vi "LHF.DB.MongoDB.vi"() -> ()   [LabVIEW 2013]
uses:
  src/LHF.DB.Mongo.lvclass
panel:
  out "Document":variant
  out "Document Part":bool
  out "error out":errorcluster
  out "Nested Documents":bool
  out "Update (Existent Field)":bool
  out "Inserted":bool
  out "Update (New Field)":bool
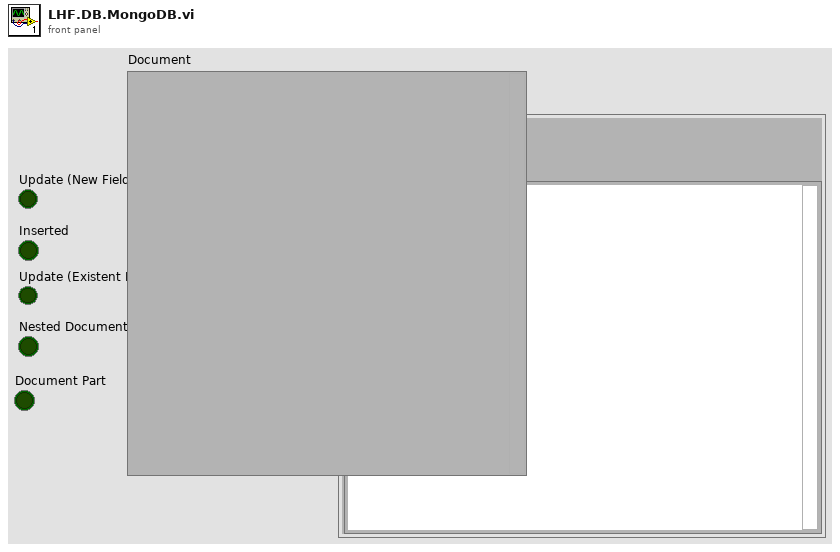
[diagram p1: front panel]
types:
  T1 = cluster{"email":string, "name":string, "status":i32, "CrazyData":cluster{"CrazyArray":cluster{"MyArray":i32[], "MyString":string, "SubSubClust":cluster{"MyArray":i32[], "MyString":string}}[][]}}
  T2 = cluster{"email":string, "name":string, "status":i32}
  T3 = cluster{"CrazyArray":cluster{"MyArray":i32[], "MyString":string, "SubSubClust":cluster{"MyArray":i32[], "MyString":string}}[][]}
  T4 = cluster{"name":string, "CrazyData":cluster{"CrazyArray":cluster{"MyArray":i32[], "MyString":string, "SubSubClust":cluster{"MyArray":i32[], "MyString":string}}[][]}}
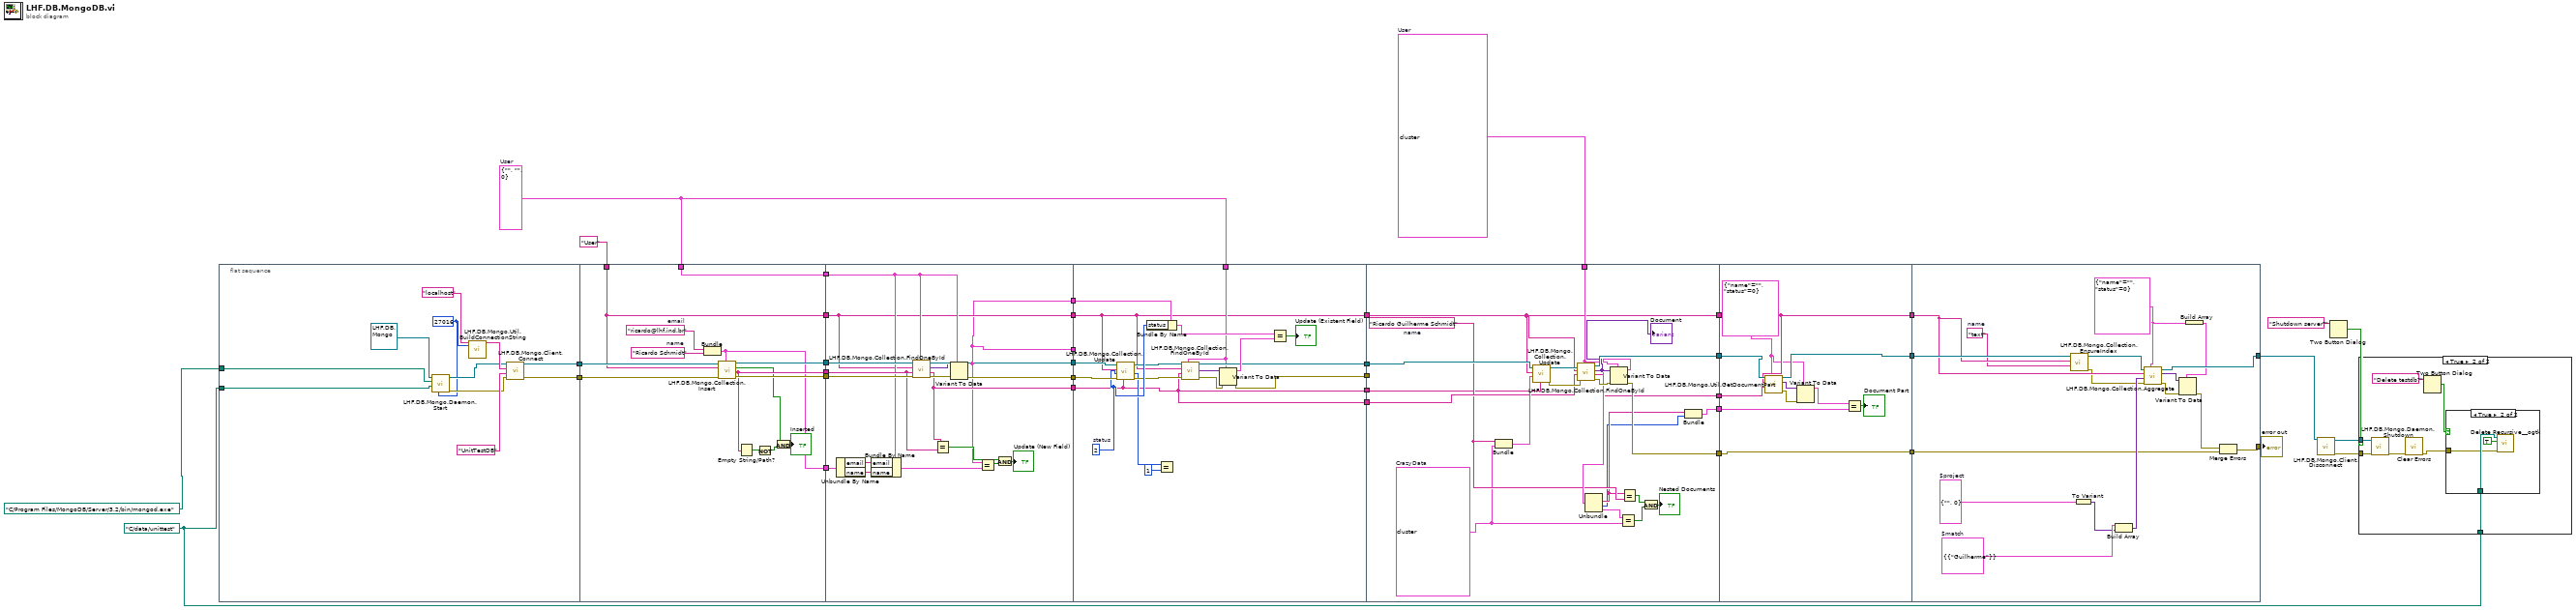
[diagram p0: block diagram]
diagram:
  w11 = path "C:/data/unittest" ("data folder")
  w17 = T1 {"email"="ricardo@lhf.ind.br", "name"="Ricardo Guilherme Schmidt", "status"=2, "CrazyData"={"CrazyArray"=[[{"MyArray"=[1, 2, 3], "MyString"="MyText", "SubSubClust"={"MyArray"=[3, 4, 5], "MyString"="MyText2"}}, {"MyArray"=[7, 8, 9], "MyString"="MyText3", "SubSubClust"={"MyArray"=[10, 11, 12], "MyString"="MyText4"}}]]}}  # User
  w22 = T2 {"email"="", "name"="", "status"=0}  # User
  n1 = flat-sequence {
    tunnel: [w46] -> w38
    tunnel: [w45] -> w37
    tunnel: w11 -> [w40]
    tunnel: path "C:/Program Files/MongoDB/Server/3.2/bin/mongod.exe" ("mongod path") -> [w39]
    tunnel: w38 -> [w61]
    tunnel: w37 -> [w63]
    tunnel: [w62] -> w36
    tunnel: [w60] -> w35
    tunnel: "User" ("database") -> [w59]
    tunnel: w22 -> [w56]
    tunnel: [w55] -> w31
    tunnel: [w59] -> w30
    tunnel: [w56] -> w29
    tunnel: [w51] -> w28
    tunnel: w36 -> [w80]
    tunnel: w35 -> [w81]
    tunnel: [w79] -> w34
    tunnel: [w76] -> w33
    tunnel: w31 -> [w75]
    tunnel: w30 -> [w66]
    tunnel: w29 -> [w73]
    tunnel: w28 -> [w74]
    tunnel: [w66] -> w27
    tunnel: [w65] -> w26
    tunnel: [w64] -> w24
    tunnel: [w64] -> w23
    tunnel: w34 -> [w98]
    tunnel: w33 -> [w99]
    tunnel: w27 -> [w83]
    tunnel: w26 -> [w82]
    tunnel: [w87] -> w25
    tunnel: w24 -> [_]
    tunnel: w23 -> [w97]
    tunnel: w22 -> [w86]
    tunnel: [w88] -> w20
    tunnel: [w82] -> w19
    tunnel: [w83] -> w18
    tunnel: [w82] -> w16
    tunnel: w25 -> [_]
    tunnel: w20 -> [w122]
    tunnel: w19 -> [w113]
    tunnel: w18 -> [w105]
    tunnel: w17 -> [w116]
    tunnel: [w118] -> w10
    tunnel: [w114] -> w8
    tunnel: [w105] -> w7
    tunnel: w16 -> [w104]
    tunnel: [w103] -> w5
    tunnel: [w100] -> w4
    tunnel: w10 -> [w133]
    tunnel: [w132] -> w9
    tunnel: w8 -> [w123]
    tunnel: w7 -> [w131]
    tunnel: [w131] -> w6
    tunnel: w5 -> [w130]
    tunnel: w4 -> [w125]
    tunnel: [w123] -> w1
    tunnel: [w149] -> w21
    tunnel: w9 -> [w150]
    tunnel: w6 -> [w139]
    tunnel: [w135] -> w13
    tunnel: w1 -> [w134]
    frame #0 {
      w41 = u32 27016 ("Port (27017)")
      n2 = call-dynamic "LHF.DB.Mongo.Daemon.Start.vi"("Port (27017)"=w41, "data folder"=w40, "mongod path"=w39, "LHF.DB.Mongo in"=refnum<class "LHF.DB.Mongo.lvclass"> refnum) -> ("error out"=w42:errorcluster, "LHF.DB.Mongo out"=w44:refnum<class "LHF.DB.Mongo.lvclass">)  [unwired: 6 in]
      n3 = call "LHF.DB.Mongo.Util.BuildConnectionString.vi"("host"="localhost", "port"=w41) -> ("connectionString"=w49:string)  [unwired: 17 in]
      n4 = call-dynamic "LHF.DB.Mongo.Client.Connect.vi"("error in (no error)"=w42, "database"="UnitTestDB", "url"=w49, "LHF.DB.Mongo in"=w44) -> ("error out"=w45:errorcluster, "LHF.DB.Mongo out"=w46:refnum<class "LHF.DB.Mongo.lvclass">)  [unwired: 6 in]
    }
    frame #1 {
      w57 = "Ricardo Schmidt"  # name
      w58 = "ricardo@lhf.ind.br"  # email
      n5 = Bundle("email"=w58, "name"=w57) -> (w51:cluster{"email":string, "name":string})  [unwired: 1 in]
      n6 = call-dynamic "LHF.DB.Mongo.Collection.Insert.vi"("Document"=w51, "error in (no error)"=w63, "Collection"=w59, "LHF.DB.Mongo"=w61) -> ("error out"=w62:errorcluster, "_id"=w55:string, "Ok"=w52:bool, "LHF.DB.Mongo out"=w60:refnum<class "LHF.DB.Mongo.lvclass">)  [unwired: 4 in]
      n7 = Empty String/Path?(string/path=w55) -> (empty?=w54:bool)
      n8 = Not(x=w54) -> (.not. x?=w53:bool)
      n9 = And(x=w52, y=w53) -> (x .and. y?=→"Inserted":bool)
    }
    frame #2 {
      n10 = Unbundle By Name(w74) -> ("email"=w72:string, "name"=w71:string)
      n11 = Bundle By Name(cluster=w73, "email"=w72, "name"=w71) -> (w70:T2)
      n12 = call-dynamic "LHF.DB.Mongo.Collection.FindOneById.vi"("type"=w73, "error in (no error)"=w80, "_id"=w75, "Collection"=w66, "LHF.DB.Mongo in"=w81) -> ("error out"=w78:errorcluster, "_id"=w65:string, "Document"=w77:variant, "LHF.DB.Mongo out"=w79:refnum<class "LHF.DB.Mongo.lvclass">)  [unwired: 3 in]
      n13 = Equal?(x=w65, y=w75) -> (x = y?=w69:bool)
      n14 = Variant To Data(error in=w78, type=w73, Variant=w77) -> (data=w64:T2, error out=w76:errorcluster)
      n15 = Equal?(x=w64, y=w70) -> (x = y?=w68:bool)
      n16 = And(x=w69, y=w68) -> (x .and. y?=→"Update (New Field)":bool)
    }
    frame #3 {
      w96 = 2  # status
      n17 = call-dynamic "LHF.DB.Mongo.Collection.Update.vi"("Query"=w82, "error in (no error)"=w99, "Update"=w96, "Collection"=w83, "LHF.DB.Mongo in"=w98) -> ("error out"=w94:errorcluster, "DocumentsAffected"=w85:i64, "LHF.DB.Mongo out"=w95:refnum<class "LHF.DB.Mongo.lvclass">)  [unwired: 3 in, 1 out]
      n18 = Bundle By Name(cluster=w97, "status"=w96) -> (w90:T2)
      n19 = Equal?(x=w85, y=i64 1) -> ()  [unwired: 1 out]
      n20 = call-dynamic "LHF.DB.Mongo.Collection.FindOneById.vi"("type"=w86, "error in (no error)"=w94, "_id"=w82, "Collection"=w83, "LHF.DB.Mongo in"=w95) -> ("error out"=w92:errorcluster, "Document"=w93:variant, "LHF.DB.Mongo out"=w88:refnum<class "LHF.DB.Mongo.lvclass">)  [unwired: 3 in, 1 out]
      n21 = Variant To Data(error in=w92, type=w86, Variant=w93) -> (data=w91:T2, error out=w87:errorcluster)
      n22 = Equal?(x=w90, y=w91) -> (x = y?=→"Update (Existent Field)":bool)
    }
    frame #4 {
      w109 = T3 {"CrazyArray"=[[{"MyArray"=[1, 2, 3], "MyString"="MyText", "SubSubClust"={"MyArray"=[3, 4, 5], "MyString"="MyText2"}}, {"MyArray"=[7, 8, 9], "MyString"="MyText3", "SubSubClust"={"MyArray"=[10, 11, 12], "MyString"="MyText4"}}], [{"MyArray"=[1, 2, 3], "MyString"="MyText", "SubSubClust"={"MyArray"=[1, 2, 3], "MyString"="MyText"}}, {"MyArray"=[1, 2, 3], "MyString"="MyText", "SubSubClust"={"MyArray"=[1, 2, 3], "MyString"="MyText"}}]]}  # CrazyData
      w111 = "Ricardo Guilherme Schmidt"  # name
      n23 = Bundle("name"=w111, "CrazyData"=w109) -> (w121:T4)  [unwired: 1 in]
      n24 = call-dynamic "LHF.DB.Mongo.Collection.Update.vi"("Query"=w104, "Update"=w121, "Collection"=w105, "LHF.DB.Mongo in"=w122) -> ("error out"=w120:errorcluster, "LHF.DB.Mongo out"=w119:refnum<class "LHF.DB.Mongo.lvclass">)  [unwired: 4 in, 2 out]
      n25 = call-dynamic "LHF.DB.Mongo.Collection.FindOneById.vi"("type"=w116, "error in (no error)"=w120, "_id"=w113, "Collection"=w105, "LHF.DB.Mongo in"=w119) -> ("error out"=w115:errorcluster, "_id"=w103:string, "Document"=w117:variant, "LHF.DB.Mongo out"=w118:refnum<class "LHF.DB.Mongo.lvclass">)  [unwired: 3 in]
      "Document" <- w117
      n26 = Variant To Data(error in=w115, type=w116, Variant=w117) -> (data=w112:T1, error out=w114:errorcluster)
      n27 = Unbundle(w112) -> ("name"=w102:string, "status"=w101:i32, "CrazyData"=w110:T3)  [unwired: 1 out]
      n28 = Equal?(x=w110, y=w109) -> (x = y?=w107:bool)
      n29 = Equal?(x=w102, y=w111) -> (x = y?=w108:bool)
      n30 = And(x=w108, y=w107) -> (x .and. y?=→"Nested Documents":bool)
      n31 = Bundle("name"=w102, "status"=w101) -> (w100:cluster{"name":string, "status":i32})  [unwired: 1 in]
    }
    frame #5 {
      w128 = cluster{"name":string, "status":i32} {"name"="", "status"=0}
      n32 = call-dynamic "LHF.DB.Mongo.Util.GetDocumentPart.vi"("projection type"=w128, "_id"=w130, "Collection"=w131, "LHF.DB.Mongo in"=w133) -> ("error out"=w127:errorcluster, "Document"=w129:variant, "LHF.DB.Mongo out"=w132:refnum<class "LHF.DB.Mongo.lvclass">)  [unwired: 4 in, 1 out]
      n33 = Variant To Data(error in=w127, type=w128, Variant=w129) -> (data=w126:cluster{"name":string, "status":i32})  [unwired: 1 out]
      n34 = Equal?(x=w126, y=w125) -> (x = y?=→"Document Part":bool)
    }
    frame #6 {
      w137 = "text"  # name
      w147 = cluster{"$text":cluster{"$search":string}} {"$text"={"$search"="Guilherme"}}  # $match
      w148 = cluster{"name":string, "status":i32} {"name"="", "status"=0}  # $project
      w143 = cluster{"name":string, "status":i32} {"name"="", "status"=0}
      n35 = call-dynamic "LHF.DB.Mongo.Collection.EnsureIndex.vi"("value"=w137, "Collection"=w139, "LHF.DB.Mongo in"=w150) -> ("error out"=w138:errorcluster, "LHF.DB.Mongo out"=w140:refnum<class "LHF.DB.Mongo.lvclass">)  [unwired: 7 in]
      n36 = To Variant(anything=w148) -> (Variant=w146:variant)
      n37 = Build Array(w147, w146) -> (w145:variant[])
      n38 = call-dynamic "LHF.DB.Mongo.Collection.Aggregate.vi"("return type"=w143, "error in (no error)"=w138, "Operations"=w145, "Collection"=w139, "LHF.DB.Mongo in"=w140) -> ("error out"=w141:errorcluster, "Documents"=w144:variant[], "LHF.DB.Mongo out"=w149:refnum<class "LHF.DB.Mongo.lvclass">)  [unwired: 3 in, 1 out]
      n39 = Build Array(w143) -> (w142:cluster{"name":string, "status":i32}[])
      n40 = Variant To Data(error in=w141, type=w142, Variant=w144) -> (error out=w136:errorcluster)  [unwired: 1 out]
      n41 = Merge Errors(w136, w134) -> (w135:errorcluster)
    }
  }
  n42 = call-dynamic "LHF.DB.Mongo.Client.Disconnect.vi"("LHF.DB.Mongo in"=w21) -> ("error out"=w15:errorcluster, "LHF.DB.Mongo out"=w14:refnum<class "LHF.DB.Mongo.lvclass">)  [unwired: 9 in]
  n43 = Two Button Dialog(message="Shutdown server?") -> (T button?=w2:bool)  [unwired: 2 in]
  n44 = case shown="True" w2 {
    tunnel: w15 -> [_ w157]
    tunnel: w14 -> [_ w156]
    tunnel: w11 -> [_ w155]
    frame False {
    }
    frame True {
      n45 = call-dynamic "LHF.DB.Mongo.Daemon.Shutdown.vi"("error in (no error)"=w157, "LHF.DB.Mongo in"=w156) -> ("error out"=w154:errorcluster)  [unwired: 8 in, 1 out]
      n46 = call <vilib>:"Clear Errors.vi"("error in (no error)"=w154) -> ("error out"=w153:errorcluster)  [unwired: 6 in]
      n47 = Two Button Dialog(message="Delete testdb?") -> (T button?=w151:bool)  [unwired: 2 in]
      n48 = case shown="True" w151 {
        tunnel: w155 -> [_ w160]
        tunnel: w153 -> [_ w158]
        frame False {
        }
        frame True {
          n49 = call <userlib>:"Delete Recursive__ogtk.vi"("error in (no error)"=w158, "Recursive? (FALSE)"=TRUE, "Path"=w160) -> ()  [unwired: 7 in, 2 out]
        }
      }
    }
  }
  "error out" <- w13
